vi "EJERCICIO _4_ESTADISTICA_CON_ARRAY.vi"() -> ()   [LabVIEW 2026]
panel:
  out "NÚMERO MIN.":dbl
  out "PROMEDIO":dbl
  out "NÚMERO MÁX.":dbl
  in  "VALORES":dbl[](array[numeric])
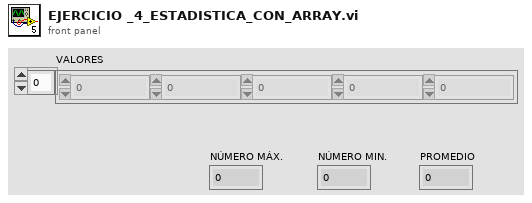
[diagram p1: front panel]
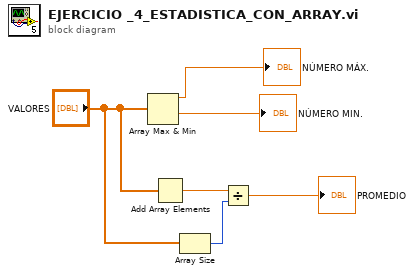
[diagram p0: block diagram]
diagram:
  n1 = Array Max & Min(array="VALORES") -> (max value=→"NÚMERO MÁX.":dbl, min value=→"NÚMERO MIN.":dbl)  [unwired: 2 out]
  n2 = Add Array Elements(numeric array="VALORES") -> (sum=w4:dbl)
  n3 = Array Size(array="VALORES") -> (size(s)=w2:i32)
  n4 = Divide(x=w4, y=w2) -> (x/y=→"PROMEDIO":dbl)
